vi "Write Data Folder.vi"(8 "error in (no error)":errorcluster, 10 "Data Folder":path, 11 "Time Entry Store-INI in":refnum<class "Time Entry Store-INI.lvclass">) -> (0 "error out":errorcluster, 3 "Time Entry Store-INI out":refnum<class "Time Entry Store-INI.lvclass">)   [LabVIEW 2024, in "Time Entry Store-INI.lvclass"]
doc: "Writes one field of this class's private data. Generated by lvai_create_accessors from the class private data control."
uses:
  Time Entry Store-INI.lvclass
  Time Entry Store-INI.lvclass/Time Entry Store-INI.ctl
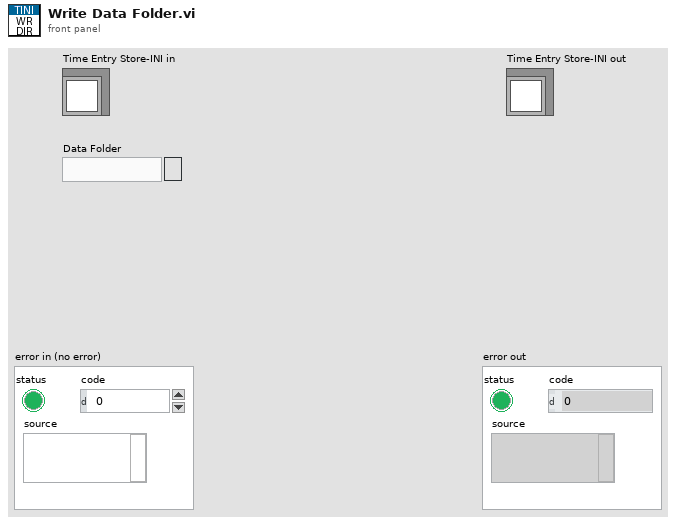
[diagram p1: front panel]
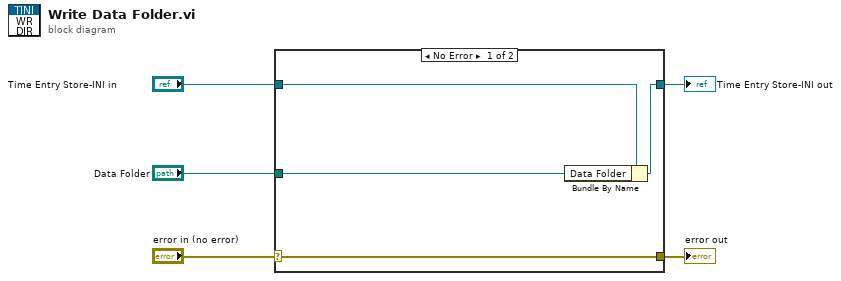
[diagram p0: block diagram]
diagram:
  n1 = case shown="No Error" "error in (no error)" {
    selector: "error in (no error)" -> [w9 w10]
    tunnel: [w9 w10] -> w4
    tunnel: [w7 w11] -> w2
    tunnel: "Time Entry Store-INI in" -> [w8 w11]
    tunnel: "Data Folder" -> [w6 _]
    frame No Error {
      n2 = Bundle By Name(cluster=w8, "Data Folder"=w6) -> (w7:refnum<class "Time Entry Store-INI.lvclass">)
    }
    frame Error {
    }
  }
  "error out" <- w4
  "Time Entry Store-INI out" <- w2
